vi "Utility - Get Icons Folder.vi"(8 "error in":errorcluster) -> (0 "error out":errorcluster, 3 "Icons Folder":path)   [LabVIEW 2014]
doc: "::: VI Helpeks :::\nCopyright (c) 2000-2026 Konstantin Shifershteyn. All rights reserved."
panel:
  # "VI Helpeks\nCopyright (c) 2012-2026 Konstantin Shifershteyn"
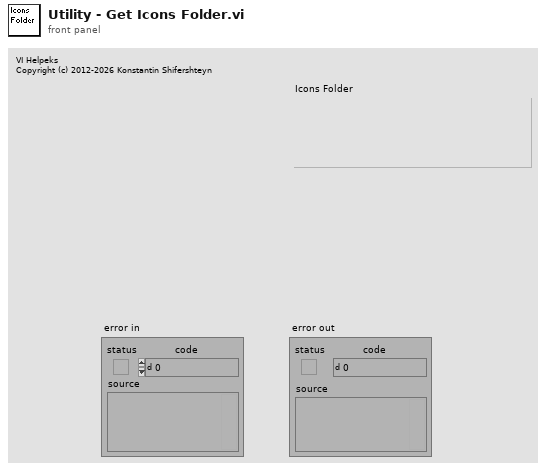
[diagram p1: front panel]
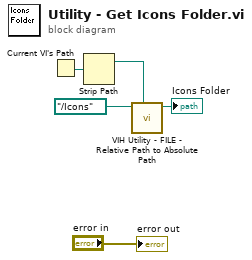
[diagram p0: block diagram]
diagram:
  n1 = Current VI's Path() -> (path=w4:path)
  n2 = Strip Path(path=w4) -> (stripped path=w3:path)  [unwired: 1 out]
  n3 = call "VIH Utility - FILE - Relative Path to Absolute Path.vi"("base path (empty: dir of Top VI)"=w3, "Path"=path "../Icons" ("base path")) -> ("Path out"=→"Icons Folder":path)  [unwired: 8 in, 1 out]
  "error out" <- "error in"
